vi "About CalcExpress.vi"   [LabVIEW 2021]
doc: "::: CalcExpress Toolkit :::\nCopyright (c) 2000-2026 Konstantin Shifershteyn. All rights reserved."
panel:
  # "CalcExpress Toolkit"
types:
  T1 = enum32{"Invalid", "Standard", "Closed", "Hidden", "Minimized", "Maximized"}
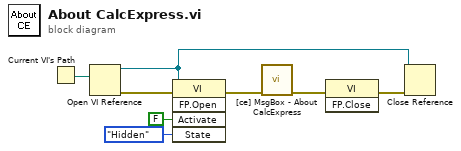
[diagram p0: block diagram]
diagram:
  n1 = Current VI's Path() -> (path=w5:path)
  n2 = Open VI Reference(vi path=w5) -> (vi reference=w6:refnum<vi>, error out=w7:errorcluster)  [unwired: 5 in]
  n3 = invoke class="VI" method="FP.Open"(reference=w6, error in=w7, "Activate"=FALSE ("Activate?"), "State"=T1."Hidden") -> (error out=w8:errorcluster)  [unwired: 1 in, 4 out]
  n4 = call "[ce] MsgBox - About CalcExpress.vi"("error in"=w8) -> ("error out"=w2:errorcluster)  [unwired: 10 in]
  n5 = invoke class="VI" method="FP.Close"(error in=w2) -> (error out=w1:errorcluster)  [unwired: 2 in, 2 out]
  n6 = Close Reference(reference=w6, error in (no error)=w1) -> ()  [unwired: 1 out]
